vi "Read CurrentPCFG.vi"(8 "Error In":errorcluster) -> (0 "Error Out":errorcluster, 1 "Config File Exists?":bool, 2 "Path Out":path)   [LabVIEW 2014, in "Standard Editor.lvlib" / "DCAF INI.lvlib"]
doc: "Read CurrentPCFG token from INI file and report whether the file exists"
uses:
  DCAF INI.lvlib
  <vilib>/Utility/config.llb/Read Key (Path).vi
  <vilib>/Utility/config.llb/NI_LVConfig.lvlib
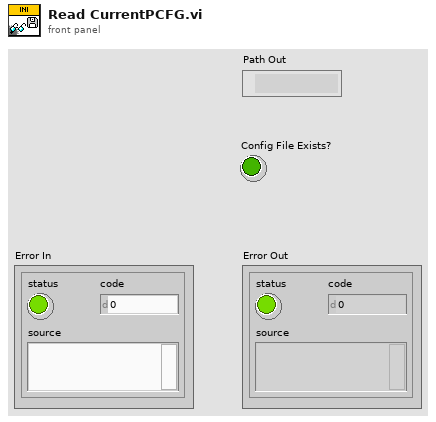
[diagram p1: front panel]
types:
  T1 = typedef "NI_LVConfig.lvlib/Config Data RefNum.ctl" = refnum<k1>
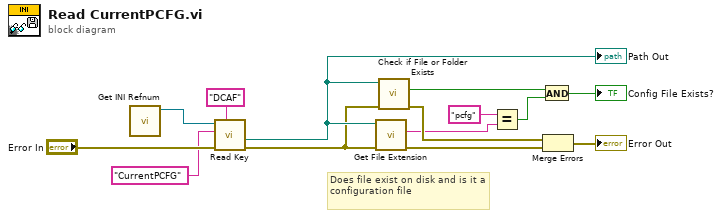
[diagram p0: block diagram]
diagram:
  # "Does file exist on disk and is it a configuration file"
  n1 = call "Get INI Refnum.vi"() -> ("INI Refnum Out"=w1:T1)  [unwired: 11 in]
  n2 = call-poly <vilib>:"Read Key.vi"("section"="DCAF", "error in (no error)"="Error In", "key"="CurrentPCFG", "refnum"=w1) -> ("error out"=w12:errorcluster, "value"=w13:path)  [unwired: 4 in, 2 out]
  "Path Out" <- w13
  n3 = call <vilib>:"Get File Extension.vi"("error in (no error)"=w12, "file"=w13) -> ("error out"=w11:errorcluster, "lowercase file extension"=w7:string)  [unwired: 6 in, 2 out]
  n4 = call <vilib>:"Check if File or Folder Exists.vi"("error in (no error)"=w12, "path"=w13) -> ("error out"=w10:errorcluster, "file or folder exists?"=w8:bool)  [unwired: 7 in, 1 out]
  n5 = Equal?(x="pcfg", y=w7) -> (x = y?=w5:bool)
  n6 = And(x=w8, y=w5) -> (x .and. y?=→"Config File Exists?":bool)
  n7 = Merge Errors(w10, w11) -> (→"Error Out":errorcluster)
